vi "read.vi"(8 "error in (no error)":errorcluster, 11 "rotationTable in":refnum<class "rotationTable.lvclass">) -> (0 "error out":errorcluster, 2 "position (°)":dbl, 3 "rotationTable out":refnum<class "rotationTable.lvclass">)   [LabVIEW 2020, in "rotationTable.lvclass"]
uses:
  rotationTable.lvclass
  lexitekDriver_client/RPC Messages/frontend_message.ctl
  lexitekDriver_client/RPC Messages/backend_response.ctl
  rotationTable.lvclass/rotationTable.ctl
  lexitekDriver_client/lexitekDriver_client.lvlib
panel:
  out "Read Data":T1
  in  "Read request":T2={"source"="lvClient::read", "command"="READ", "timestamp_ms"=0}
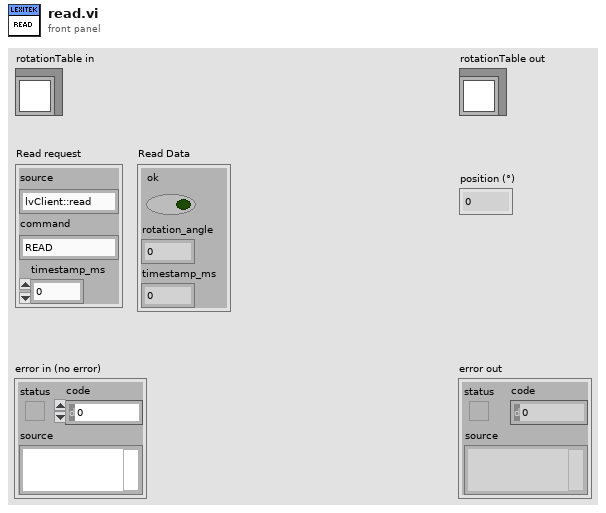
[diagram p1: front panel]
types:
  T1 = typedef "lexitekDriver_client.lvlib/backend_response.ctl" = cluster{"ok":bool, "rotation_angle":dbl, "timestamp_ms":u64}
  T2 = typedef "lexitekDriver_client.lvlib/frontend_message.ctl" = cluster{"source":string, "command":string, "timestamp_ms":u64}
  T3 = typedef "grpc-lvsupport-release.lvlib/grpcId.ctl" = u64
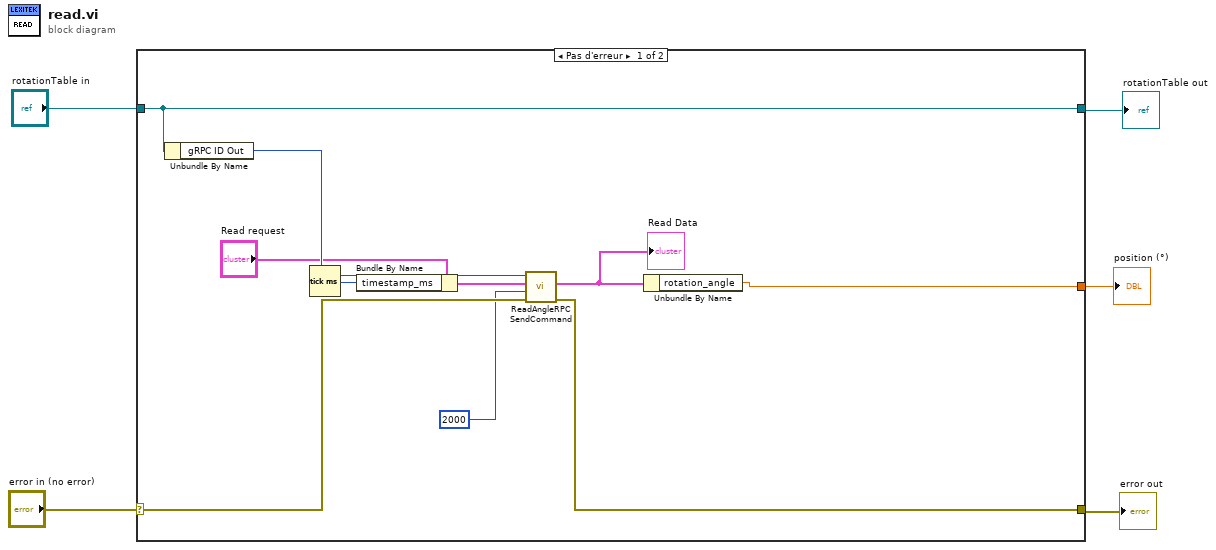
[diagram p0: block diagram]
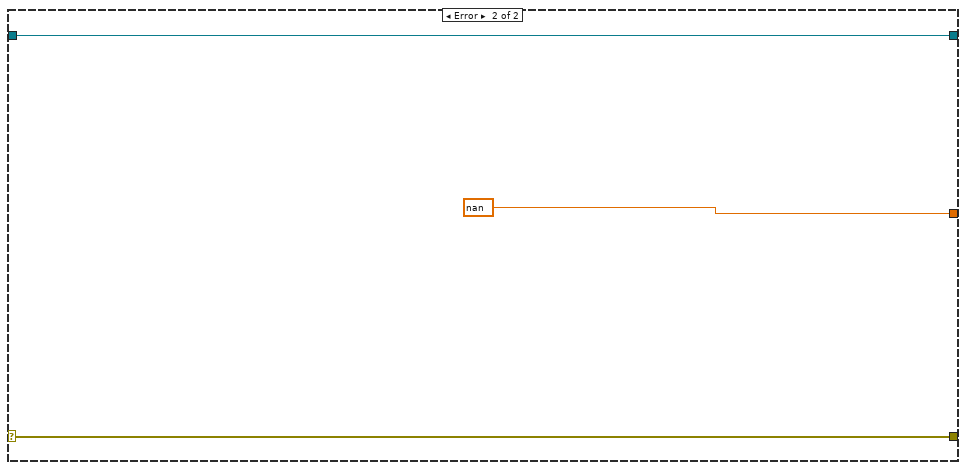
[diagram p2: hidden frame]
diagram:
  n1 = case shown="Pas d'erreur" "error in (no error)" {
    selector: "error in (no error)" -> [w14 w18]
    tunnel: [w12 w18] -> w4
    tunnel: [w15 w17] -> w2
    tunnel: "rotationTable in" -> [w15 w17]
    tunnel: [w10 nan ("rotation_angle")] -> w1
    frame No Error {
      n2 = Unbundle By Name(w15) -> ("gRPC ID Out"=w13:T3)
      n3 = Tick Count (ms)() -> (millisecond timer value=w8:u32)
      n4 = Bundle By Name(cluster="Read request", "timestamp_ms"=w8) -> (w6:T2)
      n5 = call "ReadAngleRPC SendCommand.vi"("error in"=w14, "timeout (ms)"=2000, "Request Data"=w6, "gRPC ID"=w13) -> ("error out"=w12:errorcluster, "Response Data"=w11:T1)  [unwired: 5 in, 1 out]
      "Read Data" <- w11
      n6 = Unbundle By Name(w11) -> ("rotation_angle"=w10:dbl)
    }
    frame Error {
    }
  }
  "error out" <- w4
  "rotationTable out" <- w2
  "position (°)" <- w1
